vi "Get Type String.vi"(7 "Array":bool, 8 "error in (no error)":errorcluster, 10 "Cluster or Array String":string, 11 "Cluster Info":T1[](array[typedef])) -> (0 "error out":errorcluster, 2 "elem_align":u32=8, 3 "Type String":string)   [LabVIEW 2021, in "Iceoryx.lvlib"]
uses:
  Iceoryx.lvlib
  <vilib>/CIF Foundation/CIF Utilities/DataTypes/Typedef/Cluster Info.ctl
  <vilib>/Utility/Data Type/Type Definitions/Data Type.ctl
  typedef/Errors.ctl
  Add Error Core.vi
  <vilib>/Utility/Data Type/NI_Data Type.lvlib
  <vilib>/CIF Foundation/CIF Utilities/DataTypes/DataTypes_CIF_U.lvlib
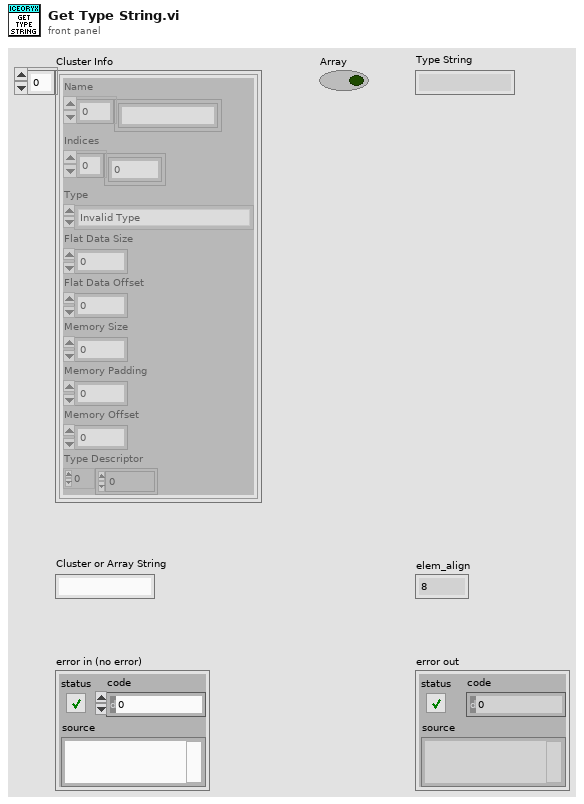
[diagram p1: front panel]
types:
  T1 = typedef "DataTypes_CIF_U.lvlib/Cluster Info.ctl" = cluster{"Name":string[], "Indices":i32[], "Type":T2, "Flat Data Size":u32, "Flat Data Offset":u32, "Memory Size":u32, "Memory Padding":u32, "Memory Offset":u32, "Type Descriptor":i16[]}
  T2 = typedef "NI_Data Type.lvlib/Data Type.ctl" = enum8{"Invalid Type", "Void", "I8", "I16", "I32", "I64", "U8", "U16", "U32", "U64", "Single Float", "Double Float", "Extended Float", "Single Complex", "Double Complex", "Extended Complex", "Enum U8", "Enum U16", "Enum U32", "Enum U64", "Single Float With Unit", "Double Float With Unit", "Extended Float With Unit", "Single Complex with Unit", "Double Complex with Unit", "Extended Complex with Unit", "Boolean", "String", "Path", "Picture", "Tag", "Array", "Cluster", "Variant", "LV Variant", "Waveform", "Timestamp", "Digital Waveform", "Digital Data", "ExpressData", "Refnum", "External Data", "VI", "Poly VI", "LabVIEW Class Instance", "Fixed Point", "Set Collection", "Map Collection"}
  T3 = typedef "Iceoryx.lvlib/Errors.ctl" = enum16{"Unsupported Type", "Empty Name", "Cluster Name"}
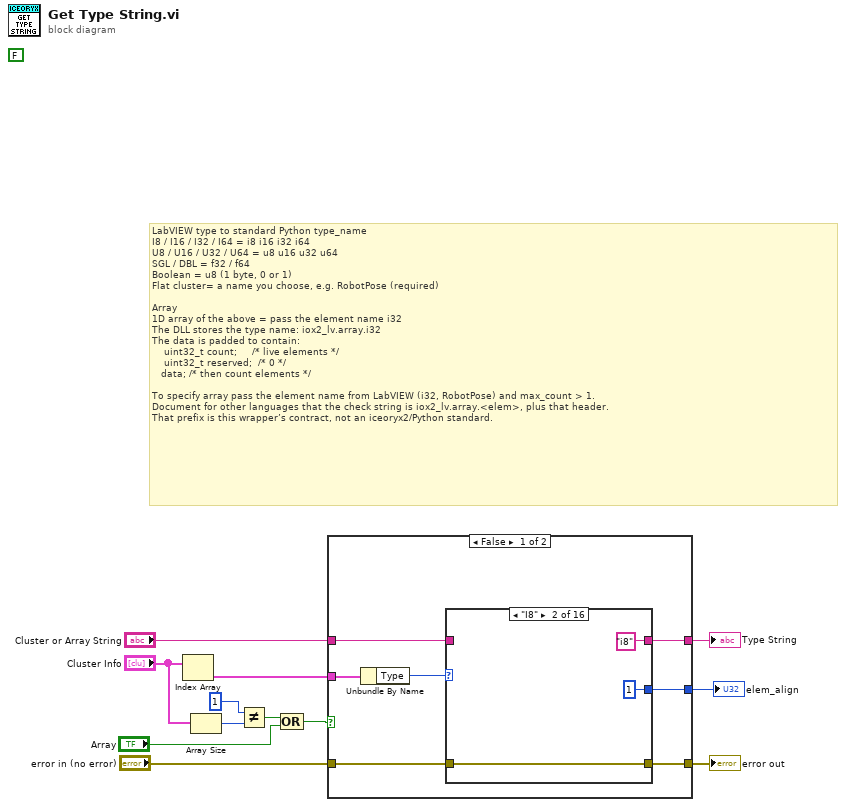
[diagram p0: block diagram]
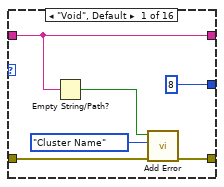
[diagram p2: hidden frame]
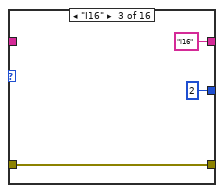
[diagram p3: hidden frame]
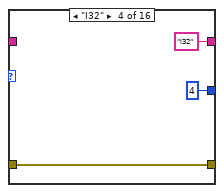
[diagram p4: hidden frame]
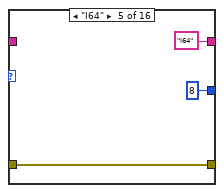
[diagram p5: hidden frame]
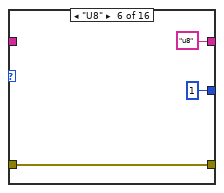
[diagram p6: hidden frame]
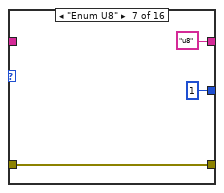
[diagram p7: hidden frame]
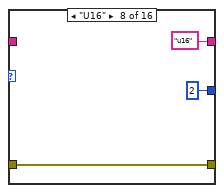
[diagram p8: hidden frame]
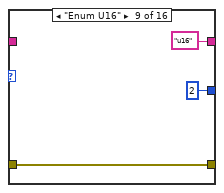
[diagram p9: hidden frame]
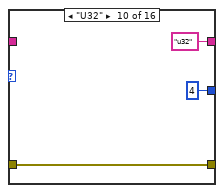
[diagram p10: hidden frame]
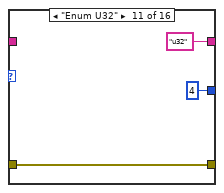
[diagram p11: hidden frame]
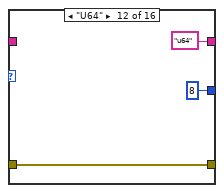
[diagram p12: hidden frame]
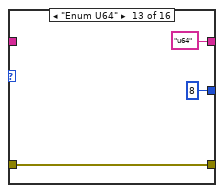
[diagram p13: hidden frame]
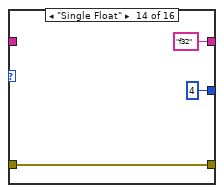
[diagram p14: hidden frame]
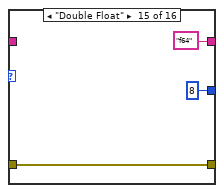
[diagram p15: hidden frame]
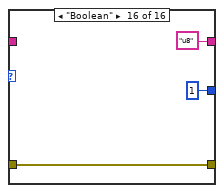
[diagram p16: hidden frame]
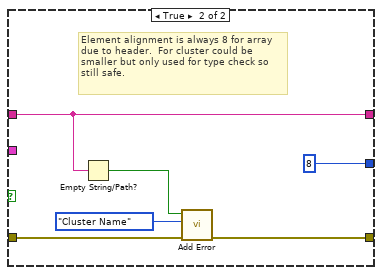
[diagram p17: hidden frame]
diagram:
  (unwired) FALSE ("Array")
  # "LabVIEW type\tto standard Python type_name\nI8 / I16 / I32 / I64 = i8 i16 i32 i64\nU8 / U16 / U32 / U64 = u8 u16 u32 u64\nSGL / DBL = f32 / f64\nBoolean = u8 (1 byte, 0 or 1)\nFlat cluster= a name you choose, e.g. RobotPose (required)\n\nArray\n1D array of the above = pass the element name i32\nThe DLL stores the type name: iox2_lv.array.i32\nThe data is padded to contain:\n    uint32_t count;     /* live elements */\n    uint32_t reserved;  /* 0 */\n   data; /* then count elements */\n\nTo specify array pass the element name from LabVIEW (i32, RobotPose) and max_count > 1. \nDocument for other languages that the check string is iox2_lv.array.<elem>, plus that header. \nThat prefix is this wrapper’s contract, not an iceoryx2/Python standard."
  n1 = Index Array(array="Cluster Info") -> (element=w11:T1)  [unwired: 1 in]
  n2 = Array Size(array="Cluster Info") -> (size(s)=w5:i32)
  n3 = Not Equal?(x=1, y=w5) -> (x != y?=w3:bool)
  n4 = Compound Arithmetic op=OR(w3, "Array") -> (w1:bool)
  n5 = case shown="False" w1 {
    tunnel: "Cluster or Array String" -> [w19 w73]
    tunnel: w11 -> [w18 _]
    tunnel: [w16 w73] -> w10
    tunnel: "error in (no error)" -> [w15 w76]
    tunnel: [w14 w75] -> w7
    tunnel: [w13 u32 8] -> w6
    frame False {
      n6 = Unbundle By Name(w18) -> ("Type"=w17:T2)
      n7 = case shown="\"I8\"" w17 {
        tunnel: [w22 "i8" "i16" "i32" "i64" "u8" "u8" "u16" "u16" "u32" "u32" "u64" "u64" "f32" "f64" "u8"] -> w16
        tunnel: w19 -> [w22 _ _ _ _ _ _ _ _ _ _ _ _ _ _ _]
        tunnel: w15 -> [w24 w27 w30 w33 w36 w39 w42 w45 w48 w51 w54 w57 w60 w63 w66 w69]
        tunnel: [w23 w27 w30 w33 w36 w39 w42 w45 w48 w51 w54 w57 w60 w63 w66 w69] -> w14
        tunnel: [u32 8 u32 1 u32 2 u32 4 u32 8 u32 1 u32 1 u32 2 u32 2 u32 4 u32 4 u32 8 u32 8 u32 4 u32 8 u32 1] -> w13
        frame "Void", Default {
          n8 = Empty String/Path?(string/path=w22) -> (empty?=w21:bool)
          n9 = call "Add Error.vi"("error in (no error)"=w24, "Error"=Errors."Cluster Name", "Insert Error"=w21) -> ("error out"=w23:errorcluster)  [unwired: 8 in]
        }
        frame "I8" {
        }
        frame "I16" {
        }
        frame "I32" {
        }
        frame "I64" {
        }
        frame "U8" {
        }
        frame "Enum U8" {
        }
        frame "U16" {
        }
        frame "Enum U16" {
        }
        frame "U32" {
        }
        frame "Enum U32" {
        }
        frame "U64" {
        }
        frame "Enum U64" {
        }
        frame "Single Float" {
        }
        frame "Double Float" {
        }
        frame "Boolean" {
        }
      }
    }
    frame True {
      # "Element alignment is always 8 for array due to header.  For cluster could be smaller but only used for type check so still safe."
      n10 = Empty String/Path?(string/path=w73) -> (empty?=w72:bool)
      n11 = call "Add Error.vi"("error in (no error)"=w76, "Error"=Errors."Cluster Name", "Insert Error"=w72) -> ("error out"=w75:errorcluster)  [unwired: 8 in]
    }
  }
  "Type String" <- w10
  "error out" <- w7
  "elem_align" <- w6
